vi "Init_log_array.vi"(10 "要创建的日志名字":string[](array[string])) -> (2 "数组":string[](array[string]))   [LabVIEW 2018, in "Log_class.lvlib"]
uses:
  Log_class.lvlib
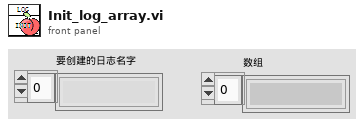
[diagram p1: front panel]
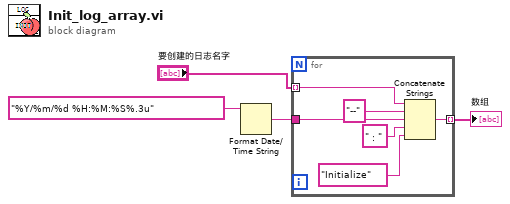
[diagram p0: block diagram]
diagram:
  n1 = Format Date/Time String(time format string (%c)="%Y/%m/%d %H:%M:%S%.3u" ("时间格式字符串(%c)")) -> (date/time string=w2:string)  [unwired: 2 in]
  n2 = for {
    tunnel: "要创建的日志名字" -> [w6] mode=indexing
    tunnel: w2 -> [w10]
    tunnel: [w7] -> w1 mode=indexing
    n3 = Concatenate Strings(w6, "--" ("字符串"), w10, "：" ("字符串"), "Initialize" ("字符串")) -> (w7:string)
  }
  "数组" <- w1
